vi "c_Spark_Close.vi"(8 "error in (no error)":errorcluster, 11 "handle":T1) -> (0 "error out":errorcluster)   [LabVIEW 2023, in "REVLibDriver.lvlib"]
uses:
  <vilib>/REVLibDriver/REVLibDriver.lvlib
  <vilib>/REV Custom Controls/c_Spark_handle.ctl
  lib/libREVLibDriver.so
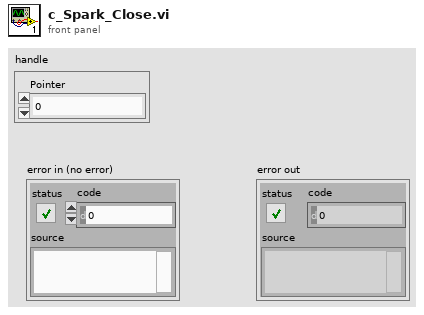
[diagram p1: front panel]
types:
  T1 = typedef "REVLibDriver.lvlib/c_Spark_handle.ctl" = cluster{"Pointer":u64}
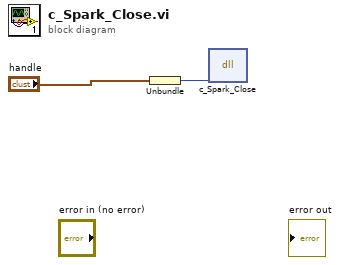
[diagram p0: block diagram]
diagram:
  n1 = Unbundle("handle") -> ("Pointer"=w1:u64)
  n2 = dll-call lib="home/systemcore/natinst/lib/libREVLibDriver.so" fn="c_Spark_Close"("handle"=w1) -> ()  [unwired: 5 in, 2 out]
